vi "Set Message Class Icon.vi"(6 "Message Type":T1, 8 "error in (no error)":errorcluster, 10 "References":T2) -> (0 "error out":errorcluster)   [LabVIEW 2023, in "Message Maker.lvclass"]
doc: "Gets the icon from the Actor class, clears it's text layer, then adds a new layer that contains the send icon Glyph. Sets this new icon to the new message class, then applys this icon to all owned items\n\nAuthor: Derek Trepanier\nCopyright: MGI 2015"
uses:
  Message Maker.lvclass
  Scripting Refs.ctl
  Message Type.ctl
  <vilib>/LabVIEW Icon API/API_Text.ctl
  <vilib>/LabVIEW Icon API/lv_icon/Controls/Layer.ctl
  <vilib>/LabVIEW Icon API/lv_icon/Classes/Layer/Layer.lvclass
  <vilib>/LabVIEW Icon API/lv_icon/Controls/LayerType.ctl
  <vilib>/LabVIEW Icon API/lv_icon/Classes/Icon/Icon.lvclass
  Message Maker.lvclass/Message Maker.ctl
  <vilib>/LabVIEW Icon API/LabVIEW Icon API.lvlib
panel:
  out "new picture":picture
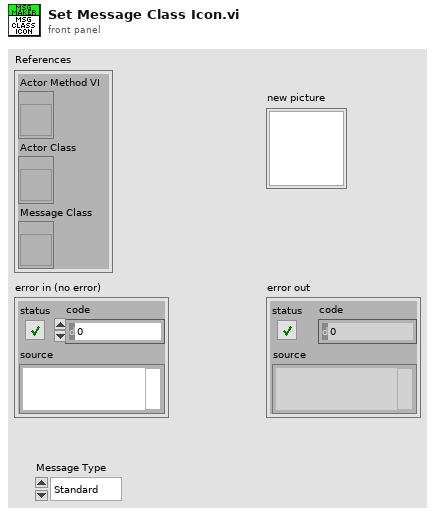
[diagram p1: front panel]
types:
  T1 = typedef "Message Maker.lvclass/Message Type.ctl" = enum16{"Standard", "Async"}
  T2 = typedef "Message Maker.lvclass/Scripting Refs.ctl" = cluster{"Actor Method VI":refnum<vi>, "Actor Class":refnum<vi>, "Message Class":refnum<vi>}
  T3 = typedef "LayerType.ctl" = enum16{"Graphic", "Text", "Tool", "Graphic Drop"}
  T4 = typedef "Layer.ctl" = cluster{"LayerIcon":picture, "LayerName":string, "Opacity":u8, "Visibility?":bool}
  T5 = typedef "LabVIEW Icon API.lvlib/API_Text.ctl" = cluster{"Line 1 text":string, "Line 2 text":string, "Line 3 text":string, "Line 4 text":string}
  T6 = typedef "imagedata.ctl" = cluster{"image type":i32, "image depth":i32, "image":u8[], "mask":u8[], "colors":u32[], "Rectangle":cluster{"left":i16, "top":i16, "right":i16, "bottom":i16}}
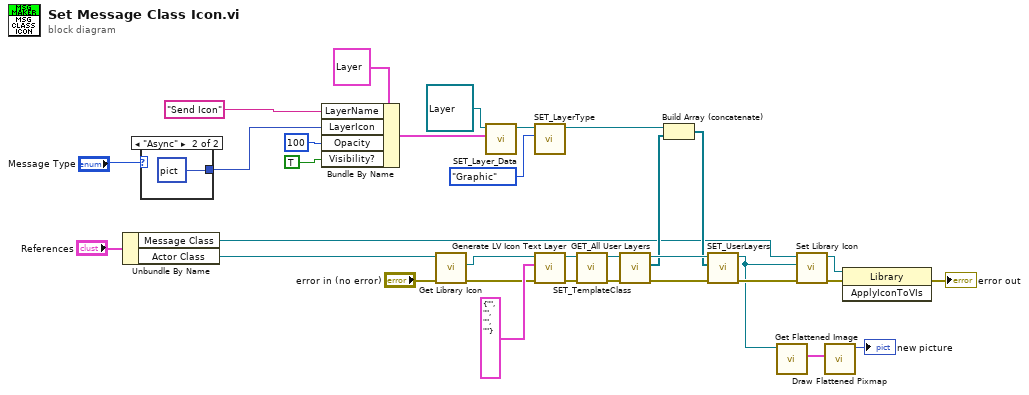
[diagram p0: block diagram]
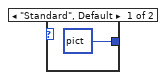
[diagram p2: hidden frame]
diagram:
  n1 = Unbundle By Name("References") -> ("Message Class"=w2:refnum<vi>, "Actor Class"=w3:refnum<vi>)
  n2 = case shown="\"Async\"" "Message Type" {
    tunnel: [picture bytes[1182] ("new picture 2") picture bytes[2464] ("new picture")] -> w8
    frame "Standard", Default {
    }
    frame "Async" {
    }
  }
  n3 = Bundle By Name(cluster=T4 {"LayerIcon"=bytes[3102], "LayerName"="", "Opacity"=100, "Visibility?"=TRUE} ("Data"), "LayerName"="Send Icon", "LayerIcon"=w8, "Opacity"=u8 100, "Visibility?"=TRUE) -> (w14:T4)
  n4 = call <vilib>:"Get Library Icon.vi"("error in (no error)"="error in (no error)", "Library Refnum in"=w3) -> ("error out"=w20:errorcluster, "Icon"=w32:refnum<class "Icon.lvclass">)  [unwired: 7 in, 1 out]
  n5 = call-dynamic "SET_Layer_Data.vi"("Data"=w14, "Layer.lvclass in"=refnum<class "Layer.lvclass"> refnum) -> ("Layer.lvclass out"=w16:refnum<class "Layer.lvclass">)  [unwired: 2 in, 7 out]
  n6 = call-dynamic "SET_LayerType.vi"("Type"=LayerType."Graphic", "Layer.lvclass in"=w16) -> ("Layer.lvclass out"=w15:refnum<class "Layer.lvclass">)  [unwired: 1 in, 8 out]
  n7 = call <vilib>:"Generate LV Icon Text Layer.vi"("error in (no error)"=w20, "Text"=T5 {"Line 1 text"="", "Line 2 text"="", "Line 3 text"="", "Line 4 text"=""}, "Icon in"=w32) -> ("error out"=w21:errorcluster, "Icon out"=w29:refnum<class "Icon.lvclass">)  [unwired: 7 in]
  n8 = call-dynamic "SET_TemplateClass.vi"("error in (no error)"=w21, "Icon.lvclass in"=w29) -> ("error out"=w22:errorcluster, "Icon.lvclass out"=w28:refnum<class "Icon.lvclass">)  [unwired: 8 in]
  n9 = call-dynamic "GET_All User Layers.vi"("error in (no error)"=w22, "Icon.lvclass in"=w28) -> ("error out"=w23:errorcluster, "User Layer"=w30:refnum<class "Layer.lvclass">[], "Icon.lvclass out"=w31:refnum<class "Icon.lvclass">)  [unwired: 7 in]
  n10 = Build Array (concatenate)(w15, w30) -> (w24:refnum<class "Layer.lvclass">[])
  n11 = call-dynamic "SET_UserLayers.vi"("error in (no error)"=w23, "Layers"=w24, "Icon.lvclass in"=w31) -> ("error out"=w25:errorcluster, "Icon.lvclass out"=w7:refnum<class "Icon.lvclass">)  [unwired: 7 in]
  n12 = call <vilib>:"Get Flattened Image.vi"("lv_icon.lvlib:Icon.lvclass in"=w7) -> ("Color Image"=w6:T6)  [unwired: 7 in, 3 out]
  n13 = call <vilib>:"Set Library Icon.vi"("error in (no error)"=w25, "Icon"=w7, "Library Refnum in"=w2) -> ("error out"=w26:errorcluster, "Library Refnum out"=w27:refnum<vi>)  [unwired: 7 in]
  n14 = call <vilib>:"Draw Flattened Pixmap.vi"("image data"=w6) -> ("new picture"=→"new picture":picture)  [unwired: 8 in]
  n15 = invoke class="Library" method="ApplyIconToVIs"(reference=w27, error in=w26) -> (error out=→"error out":errorcluster)  [unwired: 1 in, 2 out]
